vi "SeqEditor_StepMLST-cvhalfsecshow.vi"   [LabVIEW 2017]
panel:
  # "已复制！。。。"
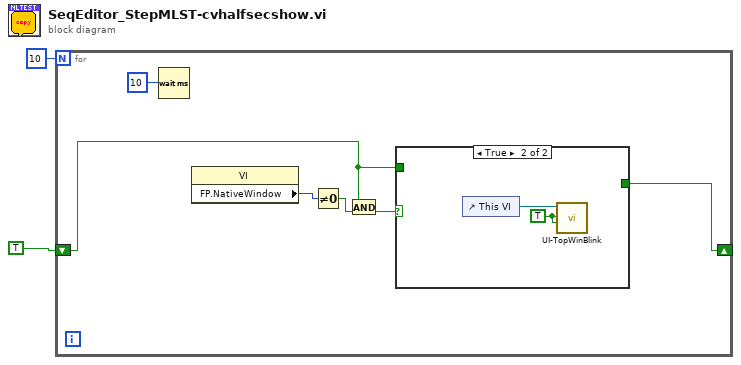
[diagram p0: block diagram]
diagram:
  n1 = for {
    N: 10 -> [_]
    shift-right: [w4] -> _
    shift-left: TRUE -> [w3]
    n2 = Wait (ms)(milliseconds to wait=u32 10) -> ()  [unwired: 1 out]
    n3 = property class="VI"() -> ("FP.NativeWindow"=w8:u64)  [unwired: 2 in, 2 out]
    n4 = Not Equal To 0?(x=w8) -> (x != 0?=w6:bool)
    n5 = And(x=w3, y=w6) -> (x .and. y?=w5:bool)
    n6 = case shown="True" w5 {
      tunnel: [w9 _] -> w4
      tunnel: w3 -> [w9 _]
      frame False {
      }
      frame True {
        w10 = TRUE ("闪烁获取焦点(T)")
        n7 = control-ref of="This VI"() -> (w11:refnum<vi>)
        n8 = call "UI-TopWinBlink.vi"("一直置顶？（F）"=w10, "闪烁获取焦点(T)"=w10, "vi ref（TopVIs）"=w11) -> ()  [unwired: 8 in, 1 out]
      }
    }
  }
